vi "ActionVIOnCompile.vi"(8 "error in (no error)":errorcluster, 11 "Device Item Ref in":T1 format="%.0x") -> (0 "error out":errorcluster)   [LabVIEW 2020, in "NI Synchronization System Explorer.lvlib"]
uses:
  NI Synchronization System Explorer.lvlib
  <vilib>/NI VeriStand/Custom Device API/Custom Device Item Ref.ctl
  Shared/Compiled Data.ctl
  Shared/Connection Settings.ctl
  Shared/Mode.ctl
  Shared/External Pin.ctl
  Shared/Routes.ctl
  Shared/Route.ctl
  Shared/Time Ref Settings.ctl
  Shared/Time Reference.ctl
  Shared/IRIG Type.ctl
  Shared/Constants.vi
  <vilib>/NI VeriStand/Custom Device API/Get Item Property (String).vi
  <vilib>/NI VeriStand/Custom Device API/Get Item Property (U16).vi
  <vilib>/NI VeriStand/Custom Device API/Get Item Property (Double).vi
  <vilib>/NI VeriStand/Custom Device API/Get Item Property (Boolean).vi
  <vilib>/NI VeriStand/Custom Device API/Set Item Property (Variant).vi
  Shared/NI Synchronization Shared.lvlib
  <vilib>/NI VeriStand/Custom Device API/Custom Device API.lvlib
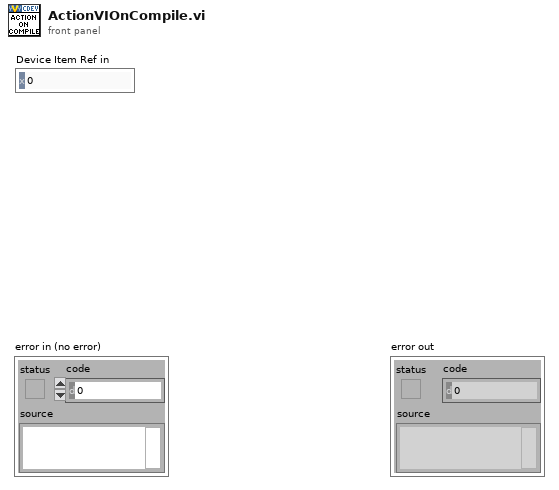
[diagram p1: front panel]
types:
  T1 = typedef "Custom Device API.lvlib/Custom Device Item Ref.ctl" = u64
  T2 = typedef "NI Synchronization Shared.lvlib/Compiled Data.ctl" = cluster{"SyncMod?":bool, "SyncMod":string, "ConnectionSettings":T3, "TimeKeeper":string, "ScanOffset(%)":dbl, "StartDelay(s)":u16, "Time Ref Settings":T8, "FIFO Locations":cluster{"BoardTime":i32[], "Status":i32[]}}
  T3 = typedef "NI Synchronization Shared.lvlib/Connection Settings.ctl" = cluster{"Mode":T4, "pxitrig":bool, "pfi0":bool, "pfi1":bool, "pfi2":bool, "External Pin":T5, "Routes":T6}
  T4 = typedef "NI Synchronization Shared.lvlib/Mode.ctl" = enum16{"Generate sample clock", "Route sample clock out of chassis", "Route sample clock into chassis", "Custom routes"}
  T5 = typedef "NI Synchronization Shared.lvlib/External Pin.ctl" = enum16{"PFI0", "PFI1", "PFI2"}
  T6 = typedef "NI Synchronization Shared.lvlib/Routes.ctl" = T7[]
  T7 = typedef "NI Synchronization Shared.lvlib/Route.ctl" = cluster{"Source":string, "Destination":string}
  T8 = typedef "NI Synchronization Shared.lvlib/Time Ref Settings.ctl" = cluster{"Time Reference":T9, "Priority 1":i32, "Priority 2":i32, "IRIG type":T10, "Terminal":string, "PPSSetTime":bool, "Start Time":timestamp}
  T9 = typedef "NI Synchronization Shared.lvlib/Time Reference.ctl" = enum16{"GPS", "IRIG", "PPS", "1588 Ordinary Clock", "802.1AS", "PXI Chassis Clock", "Free Running (Internal)"}
  T10 = typedef "NI Synchronization Shared.lvlib/IRIG Type.ctl" = enum16{"IRIGB DC", "IRIGB AM"}
  T11 = typedef "NI Synchronization Shared.lvlib/Channel.ctl" = cluster{"Name":string, "Units":string, "Default":dbl, "Description":string}
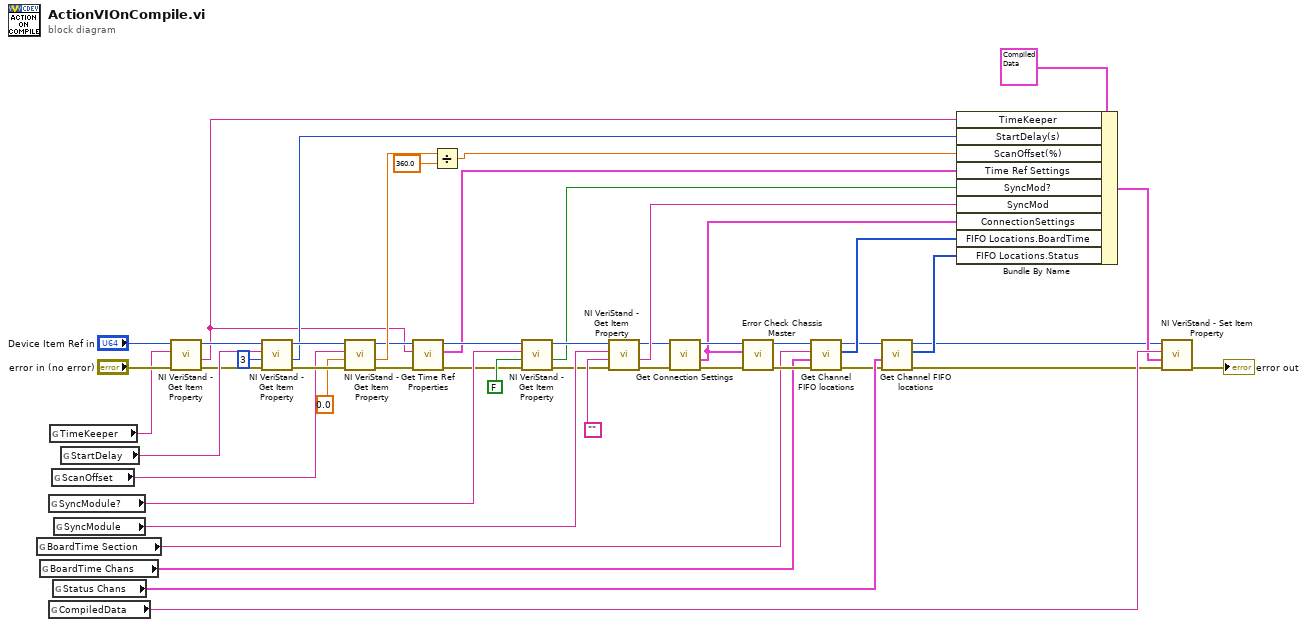
[diagram p0: block diagram]
diagram:
  n1 = global read "Constants.vi" "BoardTime Section"() -> (w9:string)
  n2 = global read "Constants.vi" "BoardTime Chans"() -> (w10:T11[])
  n3 = global read "Constants.vi" "SyncModule?"() -> (w31:string)
  n4 = global read "Constants.vi" "CompiledData"() -> (w14:string)
  n5 = global read "Constants.vi" "TimeKeeper"() -> (w47:string)
  n6 = global read "Constants.vi" "ScanOffset"() -> (w42:string)
  n7 = global read "Constants.vi" "Status Chans"() -> (w7:T11[])
  n8 = global read "Constants.vi" "SyncModule"() -> (w29:string)
  n9 = global read "Constants.vi" "StartDelay"() -> (w44:string)
  n10 = call-poly <vilib>:"NI VeriStand - Get Item Property.vi"("error in (no error)"="error in (no error)", "Property Name"=w47, "Item Ref in"="Device Item Ref in") -> ("error out"=w40:errorcluster, "Value"=w32:string, "Item Ref out"=w39:T1)  [unwired: 5 in, 1 out]
  n11 = call-poly <vilib>:"NI VeriStand - Get Item Property.vi"("error in (no error)"=w40, "Default Value"=u16 3 ("Start Offset Multiple"), "Property Name"=w44, "Item Ref in"=w39) -> ("error out"=w45:errorcluster, "Value"=w38:u16, "Item Ref out"=w46:T1)  [unwired: 4 in, 1 out]
  n12 = call-poly <vilib>:"NI VeriStand - Get Item Property.vi"("error in (no error)"=w45, "Default Value"=0.0 ("Scan Offset Scale (%)"), "Property Name"=w42, "Item Ref in"=w46) -> ("error out"=w34:errorcluster, "Value"=w37:dbl, "Item Ref out"=w33:T1)  [unwired: 4 in, 1 out]
  n13 = call "Get Time Ref Properties.vi"("error in (no error)"=w34, "TimeKeeper Module"=w32, "Device Item Ref in"=w33) -> ("error out"=w27:errorcluster, "Time Ref Settings"=w20:T8, "Item Ref out"=w26:T1)  [unwired: 6 in]
  n14 = Divide(x=w37, y=360.0) -> (x/y=w36:dbl)
  n15 = call-poly <vilib>:"NI VeriStand - Get Item Property.vi"("error in (no error)"=w27, "Default Value"=FALSE, "Property Name"=w31, "Item Ref in"=w26) -> ("error out"=w24:errorcluster, "Value"=w23:bool, "Item Ref out"=w25:T1)  [unwired: 4 in, 1 out]
  n16 = call-poly <vilib>:"NI VeriStand - Get Item Property.vi"("error in (no error)"=w24, "Default Value"="", "Property Name"=w29, "Item Ref in"=w25) -> ("error out"=w21:errorcluster, "Value"=w22:string, "Item Ref out"=w18:T1)  [unwired: 4 in, 1 out]
  n17 = call "Get Connection Settings.vi"("error in (no error)"=w21, "Item Ref in"=w18) -> ("error out"=w19:errorcluster, "Connection Settings"=w16:T3, "Item Ref out"=w17:T1)  [unwired: 6 in, 1 out]
  n18 = call "Error Check Chassis Master.vi"("error in (no error)"=w19, "Connection Settings"=w16, "Item Ref in"=w17) -> ("error out"=w12:errorcluster, "Item Ref out"=w11:T1)  [unwired: 7 in]
  n19 = call "Get Channel FIFO locations.vi"("error in (no error)"=w12, "Channels to get refs"=w10, "Section By Relative Path (\"\")"=w9, "Device Ref in"=w11) -> ("error out"=w2:errorcluster, "FIFO Locations"=w8:i32[], "Device Ref out"=w1:T1)  [unwired: 5 in]
  n20 = call "Get Channel FIFO locations.vi"("error in (no error)"=w2, "Channels to get refs"=w7, "Device Ref in"=w1) -> ("error out"=w5:errorcluster, "FIFO Locations"=w6:i32[], "Device Ref out"=w4:T1)  [unwired: 6 in]
  n21 = Bundle By Name(cluster=T2 {"SyncMod?"=FALSE, "SyncMod"="", "ConnectionSettings"={"Mode"=enum."Generate sample clock", "pxitrig"=FALSE, "pfi0"=FALSE, "pfi1"=FALSE, "pfi2"=FALSE, "External Pin"=enum."PFI0", "Routes"=[]}, "TimeKeeper"="", "ScanOffset(%)"=0.0, "StartDelay(s)"=0, "Time Ref Settings"={"Time Reference"=enum."GPS", "Priority 1"=0, "Priority 2"=0, "IRIG type"=enum."IRIGB AM", "Terminal"="", "PPSSetTime"=FALSE, "Start Time"=timestamp(0 s since 1904-01-01)}, "FIFO Locations"={"BoardTime"=[], "Status"=[]}} ("Compiled Data"), "TimeKeeper"=w32, "StartDelay(s)"=w38, "ScanOffset(%)"=w36, "Time Ref Settings"=w20, "SyncMod?"=w23, "SyncMod"=w22, "ConnectionSettings"=w16, "FIFO Locations.BoardTime"=w8, "FIFO Locations.Status"=w6) -> (w13:T2)
  n22 = call-poly <vilib>:"NI VeriStand - Set Item Property.vi"("error in (no error)"=w5, "Value"=w13, "Property Name"=w14, "Item Ref in"=w4) -> ("error out"=→"error out":errorcluster)  [unwired: 5 in, 2 out]
